vi "Pick Other Stock.vi"(11 "stock":i32) -> (3 "other":i32)   [LabVIEW 2020, in "Full Featured MCP Server.lvlib"]
doc: "Picks a random stock that is not the given one, for news and stories that need a second company."
uses:
  Full Featured MCP Server.lvlib
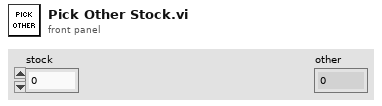
[diagram p1: front panel]
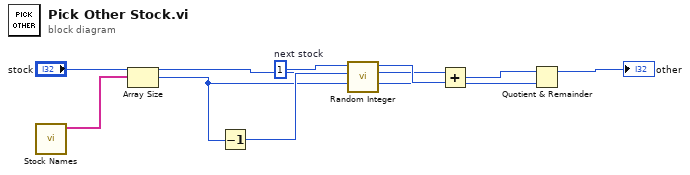
[diagram p0: block diagram]
diagram:
  w4 = 1  # next stock
  n1 = call "Stock Names.vi"() -> ("names"=w2:string[])  [unwired: 11 in]
  n2 = Array Size(array=w2) -> (size(s)=w3:i32)
  n3 = Decrement(x=w3) -> (x-1=w5:i32)
  n4 = call "Random Integer.vi"("high"=w5, "low"=w4) -> ("number"=w6:i32)  [unwired: 9 in]
  n5 = Add(x="stock", y=w6) -> (x+y=w7:i32)
  n6 = Quotient & Remainder(x=w7, y=w3) -> (x-y*floor(x/y)=→"other":i32)  [unwired: 1 out]
